vi "Test Config Iface Default Boolean.vi"(8 "error in (no error)":errorcluster, 11 "Test Case In":refnum<class "Configuration Interface Test.lvclass">) -> (0 "error out":errorcluster, 3 "Test Case Out":refnum<class "Configuration Interface Test.lvclass">)   [LabVIEW 2020, in "Configuration Interface Test.lvclass"]
uses:
  Configuration Interface Test.lvclass
  C:/Program Files (x86)/National Instruments/LabVIEW 2020/vi.lib/Astemes/LUnit/Test Case.lvclass
  source/Framework/Configuration/Configuration.lvclass
  Mock Configurable Base/Mock Configurable Base.lvclass
  <vilib>/Astemes/LUnit/Test Case.lvclass/Test Case.ctl
  Configuration Interface Test.lvclass/Configuration Interface Test.ctl
  74dde7e8-af02-4f55-b1fe-f43fb403aab3.vi
  <vilib>/Astemes/LUnit/Palette/Pass.vi
  <vilib>/Astemes/LUnit/Palette/Fail.vi
  <vilib>/Astemes/LUnit/Compare Variants.vi
  <vilib>/Astemes/LUnit/Describe Comparison.vi
  <vilib>/Astemes/LUnit/Set Assertion Type.vi
  <vilib>/Astemes/LUnit/Add test result.vi
  <vilib>/Astemes/LUnit/Variant to string.vi
  <vilib>/Astemes/LUnit/LUnit Record Assertion Result.vi
  <vilib>/Astemes/LUnit/LUnit Aggregate Assertion Results.vi
  <vilib>/Astemes/LUnit/Method Result/LUnit Merge Status.vi
  <vilib>/Astemes/LUnit/LUnit Concatenate result strings.vi
  <vilib>/Utility/Data Type/Get Type Information.vi
  <vilib>/Utility/LVClass/Get LV Class Name.vi
  <vilib>/Astemes/LUnit/Test Case.lvclass
panel:
  out "Is open?":bool
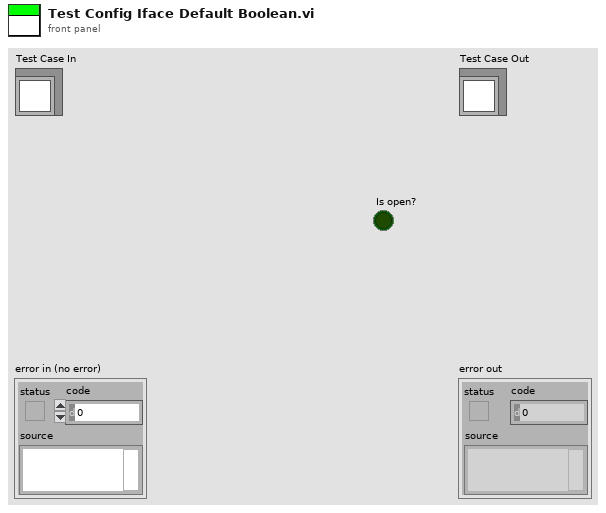
[diagram p1: front panel]
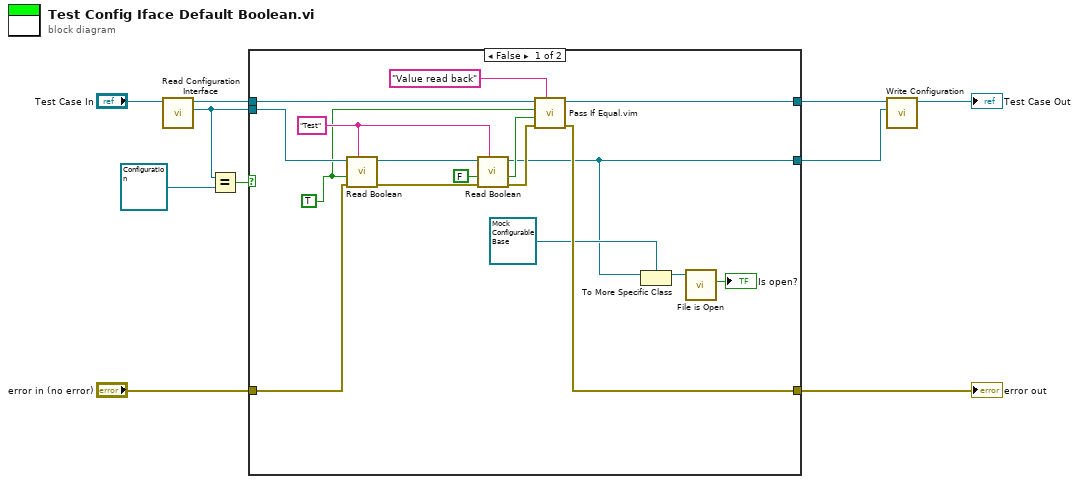
[diagram p0: block diagram]
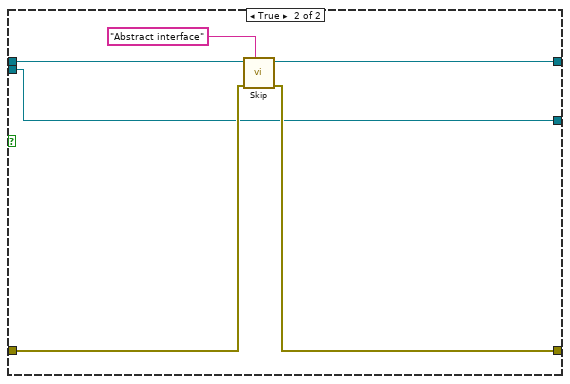
[diagram p2: hidden frame]
diagram:
  n1 = call "Read Configuration Interface.vi"("Configuration Interface Test In"="Test Case In") -> ("Configuration"=w6:refnum<class "Configuration.lvclass">, "Configuration Interface Test Out"=w8:refnum<class "Configuration Interface Test.lvclass">)  [unwired: 9 in]
  n2 = Equal?(x=w6, y=refnum<class "Configuration.lvclass"> refnum ("Configuration")) -> (x = y?=w4:bool)
  n3 = case shown="False" w4 {
    tunnel: [w16 w31] -> w9
    tunnel: w8 -> [w23 w33]
    tunnel: "error in (no error)" -> [w21 w32]
    tunnel: w6 -> [w20 w28]
    tunnel: [w12 w28] -> w3
    tunnel: [w11 w29] -> w2
    frame False {
      w18 = TRUE ("Value")
      w25 = "Test" ("key")
      n4 = call-dynamic "Read Boolean.vi"("key"=w25, "error in (no error)"=w21, "default value"=w18, "Configuration In"=w20) -> ("error out"=w26:errorcluster, "Configuration Out"=w27:refnum<class "Configuration.lvclass">)  [unwired: 5 in, 1 out]
      n5 = call-dynamic "Read Boolean.vi"("key"=w25, "error in (no error)"=w26, "default value"=FALSE, "Configuration In"=w27) -> ("error out"=w22:errorcluster, "value"=w17:bool, "Configuration Out"=w12:refnum<class "Configuration.lvclass">)  [unwired: 5 in]
      n6 = call "Pass If Equal.vim"("Description"="Value read back", "error in (no error)"=w22, "Actual"=w17, "Expected"=w18, "LUnit Test Case In"=w23) -> ("error out"=w16:errorcluster, "LUnit Test Case Out"=w11:refnum<class "Configuration Interface Test.lvclass">)  [unwired: 5 in]
      n7 = To More Specific Class(target class=refnum<class "Mock Configurable Base.lvclass"> refnum ("Mock Configurable.lvclass"), reference=w12) -> (specific class reference=w13:refnum<class "Mock Configurable Base.lvclass">)  [unwired: 1 in, 1 out]
      n8 = call "File is Open.vi"("Mock Configurable Base in"=w13) -> ("Is open?"=→"Is open?":bool)  [unwired: 8 in, 2 out]
    }
    frame True {
      n9 = call <vilib>:"Skip.vi"("Description"="Abstract interface", "error in (no error)"=w32, "LUnit Test Case In"=w33) -> ("error out"=w31:errorcluster, "LUnit Test Case Out"=w29:refnum<class "Configuration Interface Test.lvclass">)  [unwired: 7 in]
    }
  }
  "error out" <- w9
  n10 = call "Write Configuration.vi"("Configuration"=w3, "Configuration Interface Test In"=w2) -> ("Configuration Interface Test Out"=→"Test Case Out":refnum<class "Configuration Interface Test.lvclass">)  [unwired: 8 in, 1 out]
